vi "Exp curve fitting.vi"(10 "Color":T1, 11 "x (volts)":dbl) -> (3 "y (Lux)":dbl)   [LabVIEW 2020]
uses:
  controls/Color --typedef.ctl
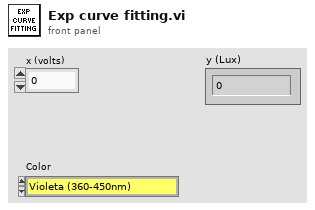
[diagram p1: front panel]
types:
  T1 = typedef "Color --typedef.ctl" = enum16{"Violeta (360-450nm)", "Azul (450-500nm)", "Verde(500-570nm)", "Amarillo (570-590nm)", "Naranja (600-610nm)", "Rojo (610-670nm)", "Blanco"}
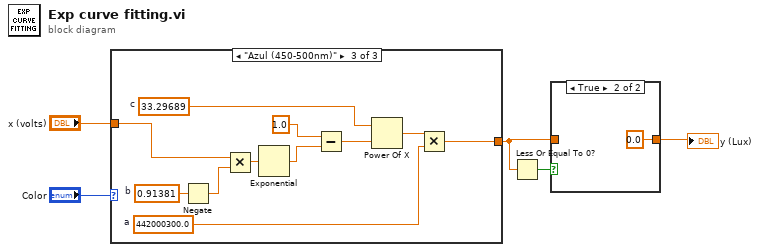
[diagram p0: block diagram]
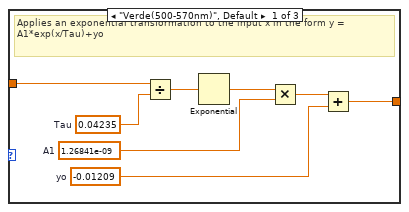
[diagram p3: hidden frame]
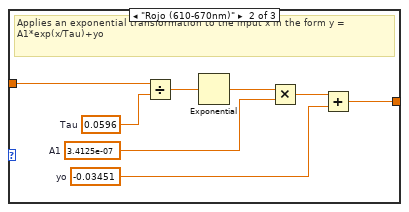
[diagram p4: hidden frame]
diagram:
  n1 = case shown="\"Azul (450-500nm)\"" "Color" {
    tunnel: "x (volts)" -> [w13 w21 w32]
    tunnel: [w6 w14 w22] -> w1
    frame "Verde(500-570nm)", Default {
      w9 = 1.26841e-09  # A1
      w7 = -0.01209  # yo
      w12 = 0.04235  # Tau
      # "Applies an exponential transformation to the input x in the form y = A1*exp(x/Tau)+yo"
      n2 = Divide(x=w13, y=w12) -> (x/y=w11:dbl)
      n3 = Exponential(1:w11) -> (0:w10:dbl)
      n4 = Multiply(x=w10, y=w9) -> (x*y=w8:dbl)
      n5 = Add(x=w8, y=w7) -> (x+y=w6:dbl)
    }
    frame "Rojo (610-670nm)" {
      w17 = 3.4125e-07  # A1
      w15 = -0.03451  # yo
      w20 = 0.0596  # Tau
      # "Applies an exponential transformation to the input x in the form y = A1*exp(x/Tau)+yo"
      n6 = Divide(x=w21, y=w20) -> (x/y=w19:dbl)
      n7 = Exponential(1:w19) -> (0:w18:dbl)
      n8 = Multiply(x=w18, y=w17) -> (x*y=w16:dbl)
      n9 = Add(x=w16, y=w15) -> (x+y=w14:dbl)
    }
    frame "Azul (450-500nm)" {
      w25 = 33.29689  # c
      w31 = 0.91381  # b
      w23 = 442000300.0  # a
      n10 = Negate(x=w31) -> (-x=w30:dbl)
      n11 = Multiply(x=w32, y=w30) -> (x*y=w29:dbl)
      n12 = Exponential(1:w29) -> (0:w28:dbl)
      n13 = Subtract(x=1.0, y=w28) -> (x-y=w26:dbl)
      n14 = Power Of X(1:w26, 2:w25) -> (0:w24:dbl)
      n15 = Multiply(x=w24, y=w23) -> (x*y=w22:dbl)
    }
  }
  n16 = Less Or Equal To 0?(x=w1) -> (x <= 0?=w3:bool)
  n17 = case shown="True" w3 {
    tunnel: [w33 0.0] -> w2
    tunnel: w1 -> [w33 _]
    frame False {
    }
    frame True {
    }
  }
  "y (Lux)" <- w2
